vi "Create.vi"(8 "error in (no error)":errorcluster, 9 "Config Hash":string, 10 "Config Version":string) -> (0 "error out":errorcluster, 3 "Config Alert Module out":refnum<class "Config Monitor Module.lvclass">)   [LabVIEW 2020, in "VolatusGUI.lvlib" / "Config Monitor Module.lvclass"]
uses:
  Config Monitor Module.lvclass
  Config Monitor Module.lvclass/Config Monitor Module.ctl
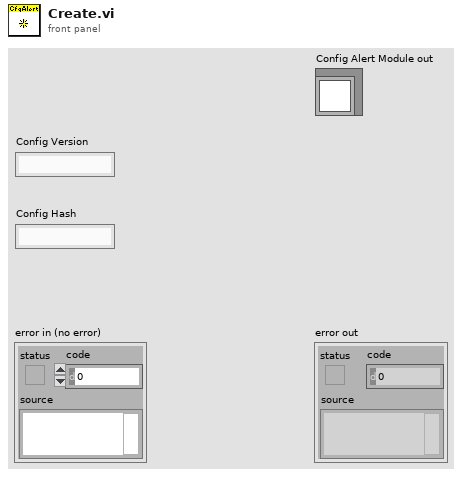
[diagram p1: front panel]
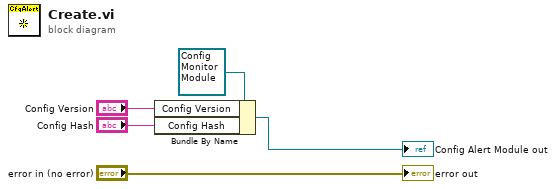
[diagram p0: block diagram]
diagram:
  n1 = Bundle By Name(cluster=refnum<class "Config Monitor Module.lvclass"> refnum ("Config Alert Module in"), "Config Version"="Config Version", "Config Hash"="Config Hash") -> (→"Config Alert Module out":refnum<class "Config Monitor Module.lvclass">)
  "error out" <- "error in (no error)"
